vi "create default channels.vi"() -> (0 "error out":errorcluster, 2 "channels":refnum<class "TBM channel.lvclass">[](array[class]), 3 "module":refnum<class "Polynomial Scale configuration.lvclass">, 5 "instance identifier":string)   [LabVIEW 2013, in "Polynomial Scale tests.lvlib"]
uses:
  Polynomial Scale tests.lvlib
  <vilib>/NI/Tag Bus Module Framework/channel/TBM channel.lvclass
  module/configuration/Polynomial Scale configuration.lvclass
  <vilib>/NI/Configuration Framework/serializable configuration/NISE_CEF_serializable configuration.lvclass
  <vilib>/NI/DCAF Templates/DCAF Scaling/module/configuration/Scaling configuration.lvclass
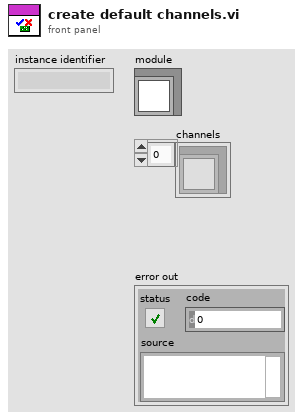
[diagram p1: front panel]
types:
  T1 = typedef "tag bus.lvlib/tag descriptor.lvclass/Data Type.ctl" = enum16{"Double", "Single", "I64", "I32", "I16", "I8", "U64", "U32", "U16", "U8", "Boolean", "String", "Array of Double", "Array of Single", "Array of I64", "Array of I32", "Array of I16", "Array of I8", "Array of U64", "Array of U32", "Array of U16", "Array of U8", "Array of Boolean", "Array of String"}
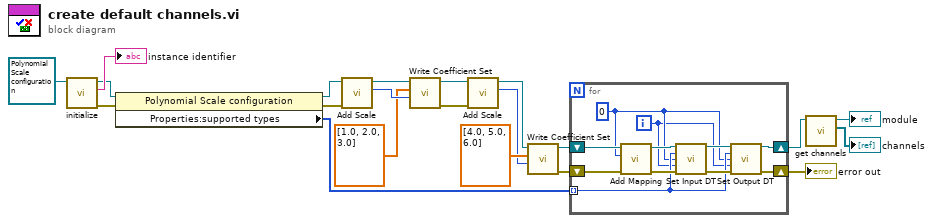
[diagram p0: block diagram]
diagram:
  n1 = call <vilib>:"initialize.vi"("configuration in"=refnum<class "Polynomial Scale configuration.lvclass"> refnum ("tag bus configurable plugin module configuration")) -> ("error out"=w20:errorcluster, "identifier"=→"instance identifier":string, "configuration out"=w19:refnum<class "Polynomial Scale configuration.lvclass">)  [unwired: 8 in]
  n2 = property class="Polynomial Scale configuration"(reference=w19, error in=w20) -> (reference out=w5:refnum<class "Polynomial Scale configuration.lvclass">, error out=w4:errorcluster, "Properties:supported types"=w9:T1[])
  n3 = call-dynamic "Add Scale.vi"("error in (no error)"=w4, "Polynomial Scale configuration in"=w5) -> ("new index"=w17:i32, "Polynomial Scale configuration out"=w16:refnum<class "Polynomial Scale configuration.lvclass">)  [unwired: 7 in, 1 out]
  n4 = call "Write Coefficient Set.vi"("scale index"=w17, "Coefficients"=dbl[] [1.0, 2.0, 3.0], "Polynomial Scale configuration in"=w16) -> ("error out"=w10:errorcluster, "Polynomial Scale configuration out"=w11:refnum<class "Polynomial Scale configuration.lvclass">)  [unwired: 7 in]
  n5 = call-dynamic "Add Scale.vi"("error in (no error)"=w10, "Polynomial Scale configuration in"=w11) -> ("new index"=w12:i32, "Polynomial Scale configuration out"=w13:refnum<class "Polynomial Scale configuration.lvclass">)  [unwired: 7 in, 1 out]
  n6 = call "Write Coefficient Set.vi"("scale index"=w12, "Coefficients"=dbl[] [4.0, 5.0, 6.0], "Polynomial Scale configuration in"=w13) -> ("error out"=w7:errorcluster, "Polynomial Scale configuration out"=w8:refnum<class "Polynomial Scale configuration.lvclass">)  [unwired: 7 in]
  n7 = for {
    tunnel: w9 -> [w24] mode=indexing
    shift-right: [w27] -> w3
    shift-left: w8 -> [w32]
    shift-right: [w28] -> w6
    shift-left: w7 -> [w31]
    i -> [w22]
    w23 = 0 ("scale index")
    n8 = call <vilib>:"Add Mapping.vi"("error in (no error)"=w31, "scale index"=w23, "Scaling configuration in"=w32) -> ("error out"=w30:errorcluster, "Scaling configuration out"=w26:refnum<class "Polynomial Scale configuration.lvclass">)  [unwired: 7 in]
    n9 = call <vilib>:"Set Input DT.vi"("Scaling configuration in"=w26, "Scale Data Type"=w24, "Scale Index"=w23, "Mapping Index"=w22, "error in (no error)"=w30) -> ("Scaling configuration out"=w25:refnum<class "Polynomial Scale configuration.lvclass">, "error out"=w29:errorcluster)  [unwired: 9 in]
    n10 = call <vilib>:"Set Output DT.vi"("Scaling configuration in"=w25, "Scale Data Type"=w24, "Scale Index"=w23, "Mapping Index"=w22, "error in (no error)"=w29) -> ("Scaling configuration out"=w27:refnum<class "Polynomial Scale configuration.lvclass">, "error out"=w28:errorcluster)  [unwired: 9 in]
  }
  "error out" <- w6
  n11 = call-dynamic "get channels.vi"("Scaling configuration in"=w3) -> ("channels"=→"channels":refnum<class "TBM channel.lvclass">[], "Scaling configuration out"=→"module":refnum<class "Polynomial Scale configuration.lvclass">)  [unwired: 9 in]
